vi "Set Button From Object.vi"(0 "Display State In":T1={"Buttons Displayed"=0, "Button States"=[], "Button Size"=0, "Button Style"=enum."Classic", "Active Button"=0, "Force Regen?"=FALSE, "Tip String Ref"=refnum}, 1 "Lazy Load?":bool=TRUE, 5 "Index (-1=at end)":i32=-1, 7 "Insert (F=Replace)":bool, 9 "Container State":T3={"Indicator?"=FALSE, "Run Mode?"=TRUE, " Refnum"=refnum}, 11 "error in (no error)":errorcluster, 12 "Button.lvclass":refnum<class "Button.lvclass">) -> (4 "Display State Out":T1={"Buttons Displayed"=0, "Button States"=[], "Button Size"=0, "Button Style"=enum."Classic", "Active Button"=0, "Force Regen?"=FALSE, "Tip String Ref"=refnum}, 15 "error out":errorcluster)   [LabVIEW 2012, in "Toolbar.xctl"]
doc: "Set the toolbar button state directly from a Button class instance"
uses:
  Toolbar.xctl
  <vilib>/_xctls/Container State.ctl
  Toolbar State.ctl
  Button_Class/Button.lvclass
  Button_Class/Type Defs/Button Style.ctl
  Button_Class/Type Defs/Button Status.ctl
  <vilib>/_xctls/XControlSupport.lvlib
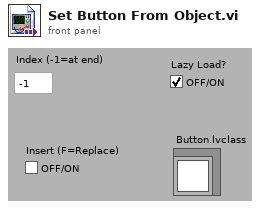
[diagram p1: front panel]
types:
  T1 = typedef "Toolbar.xctl/Toolbar State.ctl" = cluster{"Buttons Displayed":i32, "Button States":refnum<class "Button.lvclass">[], "Button Size":i32, "Button Style":T2, "Active Button":i32, "Force Regen?":bool, "Tip String Ref":refnum<vi>}
  T2 = typedef "Button.lvclass/Button Style.ctl" = enum16{"System", "Modern", "Classic", "Rounded", "Silver", "Ni Theme", "Metallic"}
  T3 = typedef "XControlSupport.lvlib/Container State.ctl" = cluster{"Indicator?":bool, "Run Mode?":bool, " Refnum":refnum<vi>}
  T4 = typedef "Button.lvclass/Button Status.ctl" = enum16{"Off", "Hover", "On", "Disabled"}
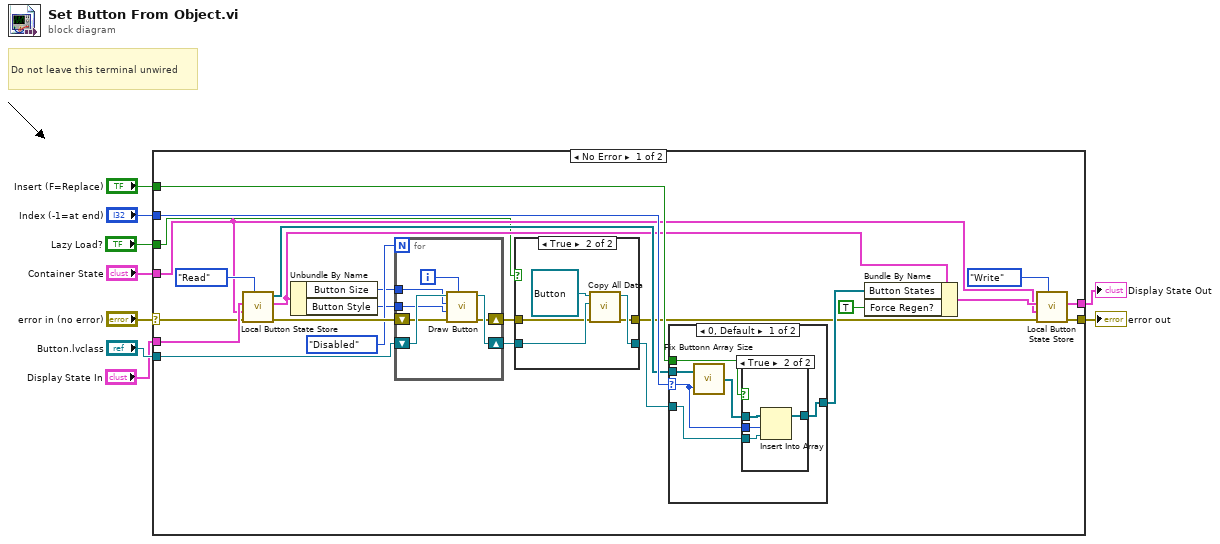
[diagram p0: block diagram]
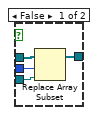
[diagram p3: hidden frame]
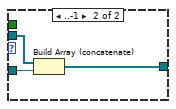
[diagram p4: hidden frame]
diagram:
  # "Do not leave this terminal unwired"
  n1 = case shown="No Error" "error in (no error)" {
    selector: "error in (no error)" -> [w21 w65]
    tunnel: "Display State In" -> [w28 w66]
    tunnel: [w25 w66] -> w8
    tunnel: [w29 w65] -> w7
    tunnel: "Index (-1=at end)" -> [w33 _]
    tunnel: "Button.lvclass" -> [w22 _]
    tunnel: "Insert (F=Replace)" -> [w32 _]
    tunnel: "Container State" -> [w24 _]
    tunnel: "Lazy Load?" -> [w14 _]
    frame No Error {
      n2 = call "Local Button State Store.vi"("Operation"=enum16{"Read", "Write"}."Read", "error in (no error)"=w21, "Container State"=w24, "Display State In"=w28) -> ("error out"=w20:errorcluster, "Display State Out"=w18:T1, "Button States"=w27:refnum<class "Button.lvclass">[])  [unwired: 5 out]
      n3 = Unbundle By Name(w18) -> ("Button Size"=w17:i32, "Button Style"=w16:T2)
      n4 = for {
        N: Button_Status."Disabled" ("Button State") -> [_]
        shift-right: [w46] -> w13
        shift-left: w22 -> [w47]
        shift-right: [w44] -> w11
        shift-left: w20 -> [w45]
        tunnel: w17 -> [w42]
        tunnel: w16 -> [w41]
        i -> [w43]
        n5 = call "Draw Button.vi"("Button State"=w43, "error in (no error)"=w45, "Button Style"=w41, "Button Size"=w42, "Button.lvclass"=w47) -> ("error out"=w44:errorcluster, "Button.lvclass Out"=w46:refnum<class "Button.lvclass">)  [unwired: 1 in, 4 out]
      }
      n6 = case shown="True" w14 {
        tunnel: w13 -> [w35 w39]
        tunnel: [w35 w38] -> w12
        tunnel: w11 -> [w34 w37]
        tunnel: [w34 w36] -> w10
        frame False {
        }
        frame True {
          n7 = call-dynamic "Copy All Data.vi"("error in (no error)"=w37, "src"=w39, "dest"=refnum<class "Button.lvclass"> refnum) -> ("error out"=w36:errorcluster, "object out"=w38:refnum<class "Button.lvclass">)  [unwired: 7 in]
        }
      }
      n8 = case shown="0, Default" w33 {
        selector: w33 -> [w51 _]
        tunnel: w27 -> [w48 w64]
        tunnel: w12 -> [w50 w63]
        tunnel: [w49 w62] -> w15
        tunnel: w32 -> [w53 _]
        frame 0, Default {
          n9 = call "Fix Buttonn Array Size.vi"("Number of Buttons"=w51, "Button States In"=w48) -> ("Button States Out"=w52:refnum<class "Button.lvclass">[])
          n10 = case shown="True" w53 {
            tunnel: w52 -> [w57 w61]
            tunnel: w51 -> [w56 w59]
            tunnel: w50 -> [w55 w60]
            tunnel: [w54 w58] -> w49
            frame False {
              n11 = Replace Array Subset(array=w57, new element=w55, index=w56) -> (w54:refnum<class "Button.lvclass">[])
            }
            frame True {
              n12 = Insert Into Array(array=w61, index=w59, new element=w60) -> (w58:refnum<class "Button.lvclass">[])
            }
          }
        }
        frame ..-1 {
          n13 = Build Array (concatenate)(w64, w63) -> (w62:refnum<class "Button.lvclass">[])
        }
      }
      n14 = Bundle By Name(cluster=w18, "Button States"=w15, "Force Regen?"=TRUE) -> (w26:T1)
      n15 = call "Local Button State Store.vi"("Operation"=enum16{"Read", "Write"}."Write", "error in (no error)"=w10, "Container State"=w24, "Display State In"=w26) -> ("error out"=w29:errorcluster, "Display State Out"=w25:T1)  [unwired: 1 in, 5 out]
    }
    frame Error {
    }
  }
  "Display State Out" <- w8
  "error out" <- w7
